vi "COMPOUND ARTHEMETIC.vi"() -> ()   [LabVIEW 2021]
panel:
  out "Boolean 3":bool
  in  "Boolean 2":bool
  in  "Boolean 5":bool
  in  "Boolean 4":bool
  in  "Boolean":bool
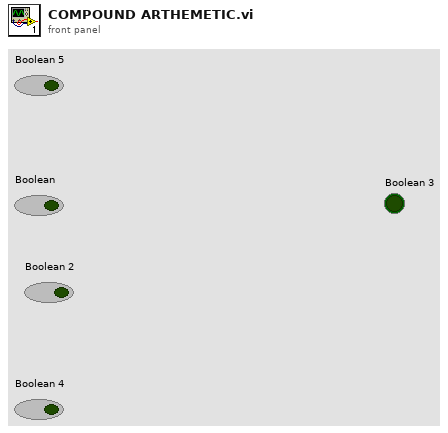
[diagram p1: front panel]
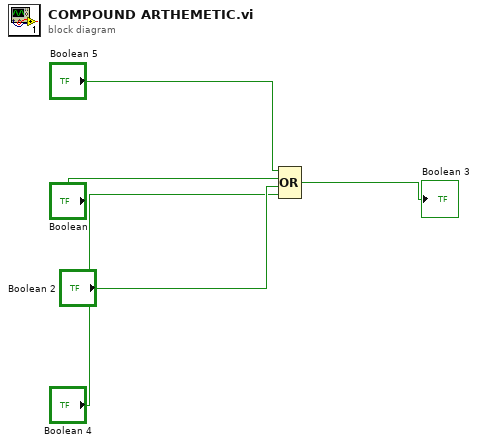
[diagram p0: block diagram]
diagram:
  n1 = Compound Arithmetic op=OR("Boolean 5", "Boolean", "Boolean 2", "Boolean 4") -> (→"Boolean 3":bool)
